vi "Determine Listbox Values.vi"(8 "error in (no error)":errorcluster, 11 "SE UI cluster in":T1={"Node Ptr"=18446744073709551615, "Add"=refnum, "Remove"=refnum, "Registers ListBox"=refnum} {"Node Ptr" format="%.0x"}) -> (0 "error out":errorcluster, 1 "Not imported item Indexes":i32[](array[numeric]), 2 "Selected item indexes":i32[](array[numeric]), 3 "SE UI cluster out":T1={"Node Ptr"=18446744073709551615, "Add"=refnum, "Remove"=refnum, "Registers ListBox"=refnum} {"Node Ptr" format="%.0x"})   [LabVIEW 2020, in "FPGA Addon System Explorer.lvlib"]
uses:
  FPGA Addon System Explorer.lvlib
  Types/SE UI Cluster.ctl
  <vilib>/NI VeriStand/Custom Device API/Custom Device Item Ref.ctl
  Addon Shared/Types/FG Action.ctl
  <vilib>/Utility/miscctls.llb/LVRowAndColumnUnsignedTypeDef.ctl
  Addon Shared/SubVIs/Constants.vi
  <vilib>/NI/NI VeriStand Advanced SysDef API/SysDef API/SysDef.Property.Get.vi
  <vilib>/NI/NI VeriStand Advanced SysDef API/_SubVIs/SysDef.Property.Get.Variant.vi
  <vilib>/NI/NI VeriStand Advanced SysDef API/SysDef API/SysDef.Property.Set.vi
  <vilib>/NI/NI VeriStand Advanced SysDef API/_SubVIs/SysDef.Property.Set.Variant.vi
  Addon Shared/FPGA Addon Shared.lvlib
  <vilib>/NI VeriStand/Custom Device API/Custom Device API.lvlib
  APIs/Scripting API/Scripting API.lvlib
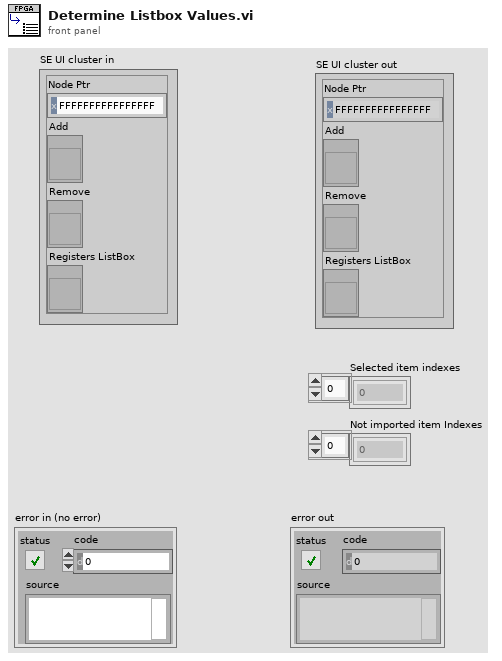
[diagram p1: front panel]
types:
  T1 = typedef "FPGA Addon System Explorer.lvlib/SE UI Cluster.ctl" = cluster{"Node Ptr":T2, "Add":refnum<vi>, "Remove":refnum<vi>, "Registers ListBox":refnum<vi>}
  T2 = typedef "Custom Device API.lvlib/Custom Device Item Ref.ctl" = u64
  T3 = typedef "FPGA Addon Shared.lvlib/FG Action.ctl" = enum8{"GET", "SET"}
  T4 = typedef "LVRowAndColumnUnsignedTypeDef.ctl" = cluster{"Row":u32, "Column":u32}
  T5 = typedef "FPGA Addon Shared.lvlib/Register Information.ctl" = cluster{"Name":string, "Data Type":T6, "Default Value":variant, "Attributes":variant}
  T6 = typedef "FPGA Addon Shared.lvlib/FPGA Addon Data Type.ctl" = enum8{"<Null>", "I8", "I16", "I32", "I64", "U8", "U16", "U32", "U64", "SGL", "Boolean", "Analog PWM In Settings", "Analog PWM In", "Digital PWM In Settings", "Digital PWM In", "Digital PWM Out", "Sine Out", "FXP", "FXP+/-24.5", "FXP+/-16.5", "FXP+/-32.8", "FXP+/-64.32", "FXP+/-16.7", "FXP+/-20.5", "FXP+/-27.5", "FXP+/-32.16", "FXP+16.3", "FXP+18.3", "Digital Static In", "Digital Static Out", "Digital Static In Settings", "Digital WSS Out", "Quad Encoder Settings", "Quad Encoder In", "Group"}
  T7 = typedef "FPGA Addon Shared.lvlib/DMA Information.ctl" = cluster{"Name":string, "Data Type":T6}
  T8 = typedef "Custom Device API.lvlib/Custom Device Item Info.ctl" = cluster{"Name":string, "Is Channel":bool, "GUID":string, "Is Waveform":bool}
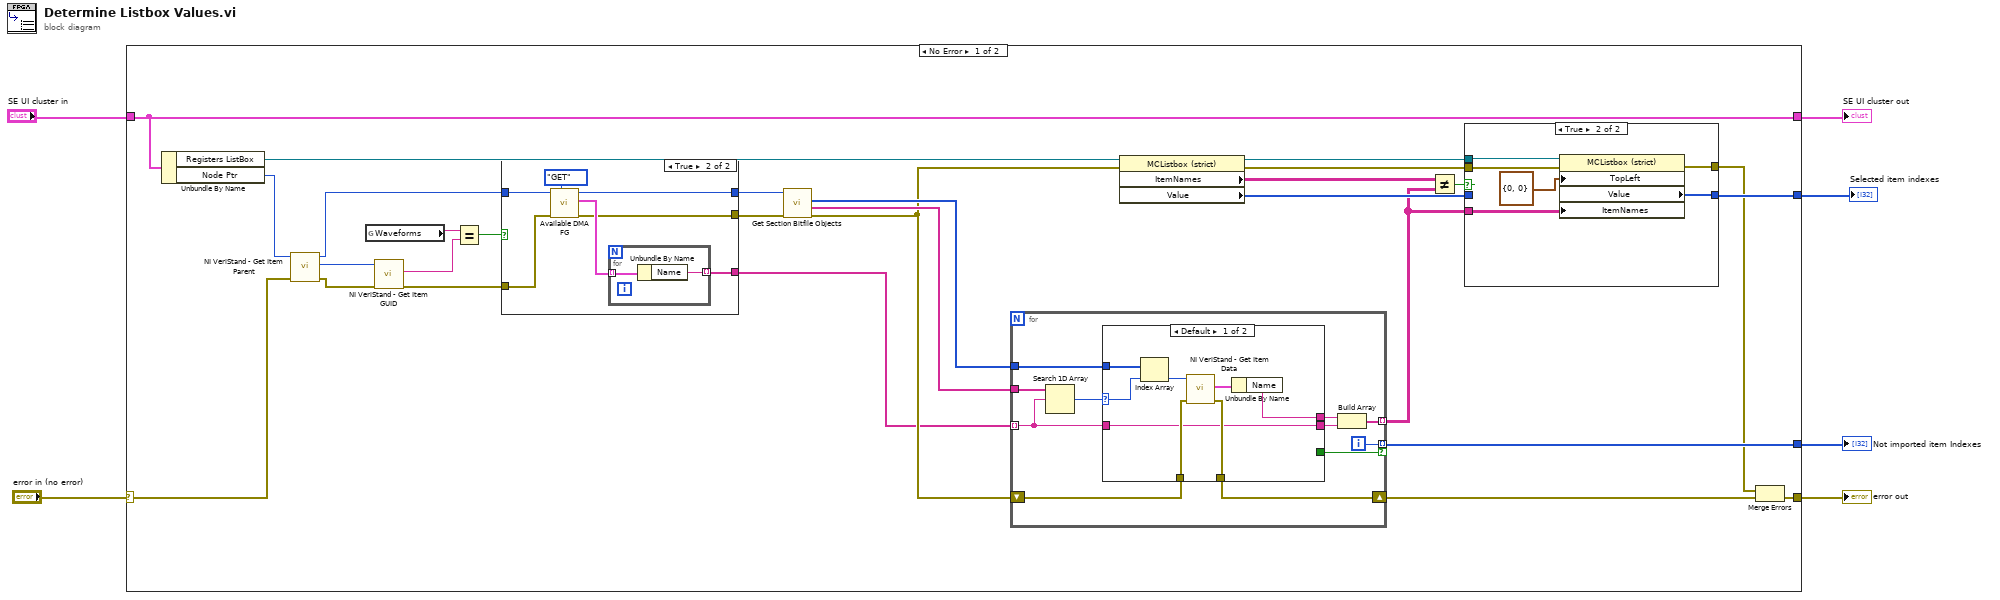
[diagram p0: block diagram]
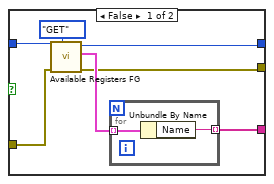
[diagram p2: hidden frame]
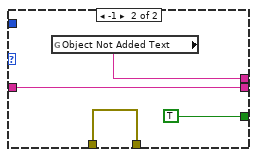
[diagram p4: hidden frame]
diagram:
  n1 = case shown="No Error" "error in (no error)" {
    selector: "error in (no error)" -> [w15 w85]
    tunnel: [w34 _] -> w6
    tunnel: [w20 w85] -> w5
    tunnel: "SE UI cluster in" -> [w31 w84]
    tunnel: [w31 w84] -> w2
    tunnel: [w30 _] -> w1
    frame No Error {
      n2 = Unbundle By Name(w31) -> ("Registers ListBox"=w29:refnum<vi>, "Node Ptr"=w18:T2)
      n3 = call <vilib>:"NI VeriStand - Get Item Parent.vi"("error in (no error)"=w15, "Item Ref in"=w18) -> ("error out"=w16:errorcluster, "Parent Ref"=w17:T2, "Item Ref out"=w13:T2)  [unwired: 6 in, 1 out]
      n4 = global read "Constants.vi" "Waveforms"() -> (w11:string)
      n5 = call <vilib>:"NI VeriStand - Get Item GUID.vi"("error in (no error)"=w16, "Item Ref in"=w17) -> ("error out"=w10:errorcluster, "GUID"=w12:string)  [unwired: 7 in, 1 out]
      n6 = Equal?(x=w11, y=w12) -> (x = y?=w14:bool)
      n7 = case shown="True" w14 {
        tunnel: w13 -> [w40 w50]
        tunnel: w10 -> [w36 w49]
        tunnel: [w39 w46] -> w9
        tunnel: [w37 w45] -> w7
        tunnel: [w35 w44] -> w8
        frame False {
          n8 = call "Available Registers FG.vi"("Action"=FG_Action."GET", "error in (no error)"=w36, "Item Ref"=w40) -> ("error out"=w35:errorcluster, "Available Registers"=w38:T5[], "Item Ref out"=w39:T2)  [unwired: 6 in]
          n9 = for {
            tunnel: [w43] -> w37 mode=indexing
            tunnel: w38 -> [w42] mode=indexing
            n10 = Unbundle By Name(w42) -> ("Name"=w43:string)
          }
        }
        frame True {
          n11 = call "Available DMA FG.vi"("Action"=FG_Action."GET", "error in (no error)"=w49, "Item Ref"=w50) -> ("error out"=w44:errorcluster, "Available DMA"=w47:T7[], "Item Ref out"=w46:T2)  [unwired: 6 in]
          n12 = for {
            tunnel: w47 -> [w52] mode=indexing
            tunnel: [w51] -> w45 mode=indexing
            n13 = Unbundle By Name(w52) -> ("Name"=w51:string)
          }
        }
      }
      n14 = call "Get Section Bitfile Objects.vi"("error in"=w8, "item ref in"=w9) -> ("error out"=w23:errorcluster, "bitfile object names"=w33:string[], "section children refs"=w32:T2[])  [unwired: 6 in, 1 out]
      n15 = for {
        tunnel: [w69] -> w24 mode=indexing
        tunnel: [w68] -> w34 mode=indexing if=w67
        tunnel: w33 -> [w66]
        tunnel: w32 -> [w65]
        shift-right: [w63] -> w21
        shift-left: w23 -> [w64]
        tunnel: w7 -> [w62] mode=indexing
        i -> [w68]
        n16 = Search 1D Array(1D array=w66, element=w62) -> (index of element=w71:i32)  [unwired: 1 in]
        n17 = case shown="Default" w71 {
          selector: w71 -> [w79 _]
          tunnel: [w75 w82] -> w70
          tunnel: [_ TRUE] -> w67
          tunnel: w65 -> [w78 _]
          tunnel: w64 -> [w74 w81]
          tunnel: [w73 w81] -> w63
          tunnel: w62 -> [w72 w80]
          tunnel: [w72 w80] -> w61
          frame Default {
            n18 = Index Array(array=w78, index=w79) -> (element=w76:T2)
            n19 = call <vilib>:"NI VeriStand - Get Item Data.vi"("error in (no error)"=w74, "Item Ref in"=w76) -> ("error out"=w73:errorcluster, "Item Info"=w77:T8)  [unwired: 6 in, 2 out]
            n20 = Unbundle By Name(w77) -> ("Name"=w75:string)
          }
          frame -1 {
            n21 = global read "Constants.vi" "Object Not Added Text"() -> (w82:string)
          }
        }
        n22 = Build Array(w70, w61) -> (w69:string[])
      }
      n23 = property class="MCListbox (strict)"(reference=w29, error in=w23) -> (reference out=w28:refnum<vi>, error out=w22:errorcluster, "ItemNames"=w27:string[][], "Value"=w25:i32[])
      n24 = Not Equal?(x=w27, y=w24) -> (x != y?=w26:bool)
      n25 = case shown="True" w26 {
        tunnel: [w54 w59] -> w30
        tunnel: w28 -> [_ w60]
        tunnel: w25 -> [w54 _]
        tunnel: w24 -> [_ w58]
        tunnel: w22 -> [w53 w56]
        tunnel: [w53 w55] -> w19
        frame False {
        }
        frame True {
          n26 = property class="MCListbox (strict)"(reference=w60, error in=w56, "TopLeft"=T4 {"Row"=0, "Column"=0} ("Top Left Visible Cell"), "ItemNames"=w58) -> (error out=w55:errorcluster, "Value"=w59:i32[])  [unwired: 1 out]
        }
      }
      n27 = Merge Errors(w19, w21) -> (w20:errorcluster)
    }
    frame Error {
    }
  }
  "error out" <- w5
  "Not imported item Indexes" <- w6
  "SE UI cluster out" <- w2
  "Selected item indexes" <- w1
